vi "Migrate Common Dependencies.vi"(0 "project path":path, 5 "measurement path":path, 7 "dependencies path":path[](array[path]), 11 "error in":errorcluster) -> (4 "project reference":refnum<vi>, 6 "measurement core reference":refnum<vi>, 8 "outside items":string[](array[string]), 10 "library":T1[](array[typedef]), 15 "error out":errorcluster)   [LabVIEW 2021, in "Multiple Converter.lvlib"]
uses:
  Multiple Converter.lvlib
  TypeDefs/Library Info.ctl
  Path Functions/Path Functions.lvlib
  Converter Reusables/Converter Reusables.lvlib
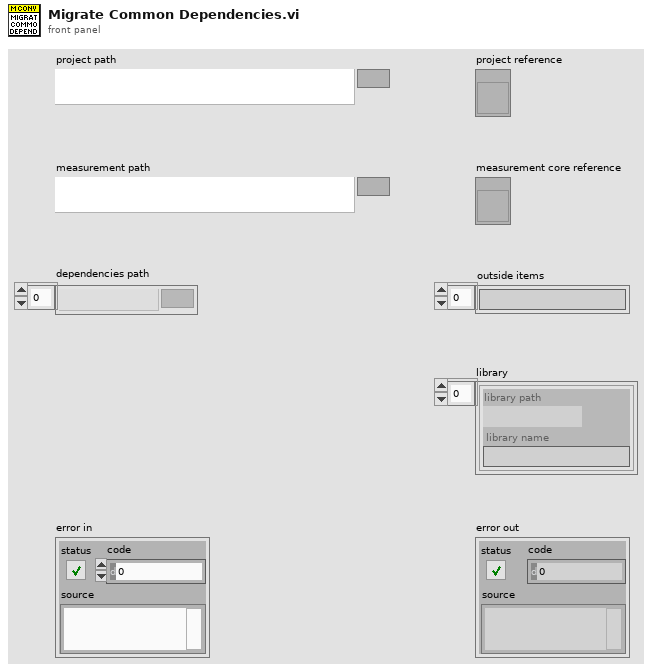
[diagram p1: front panel]
types:
  T1 = typedef "Multiple Converter.lvlib/Library Info.ctl" = cluster{"library path":path, "library name":string}
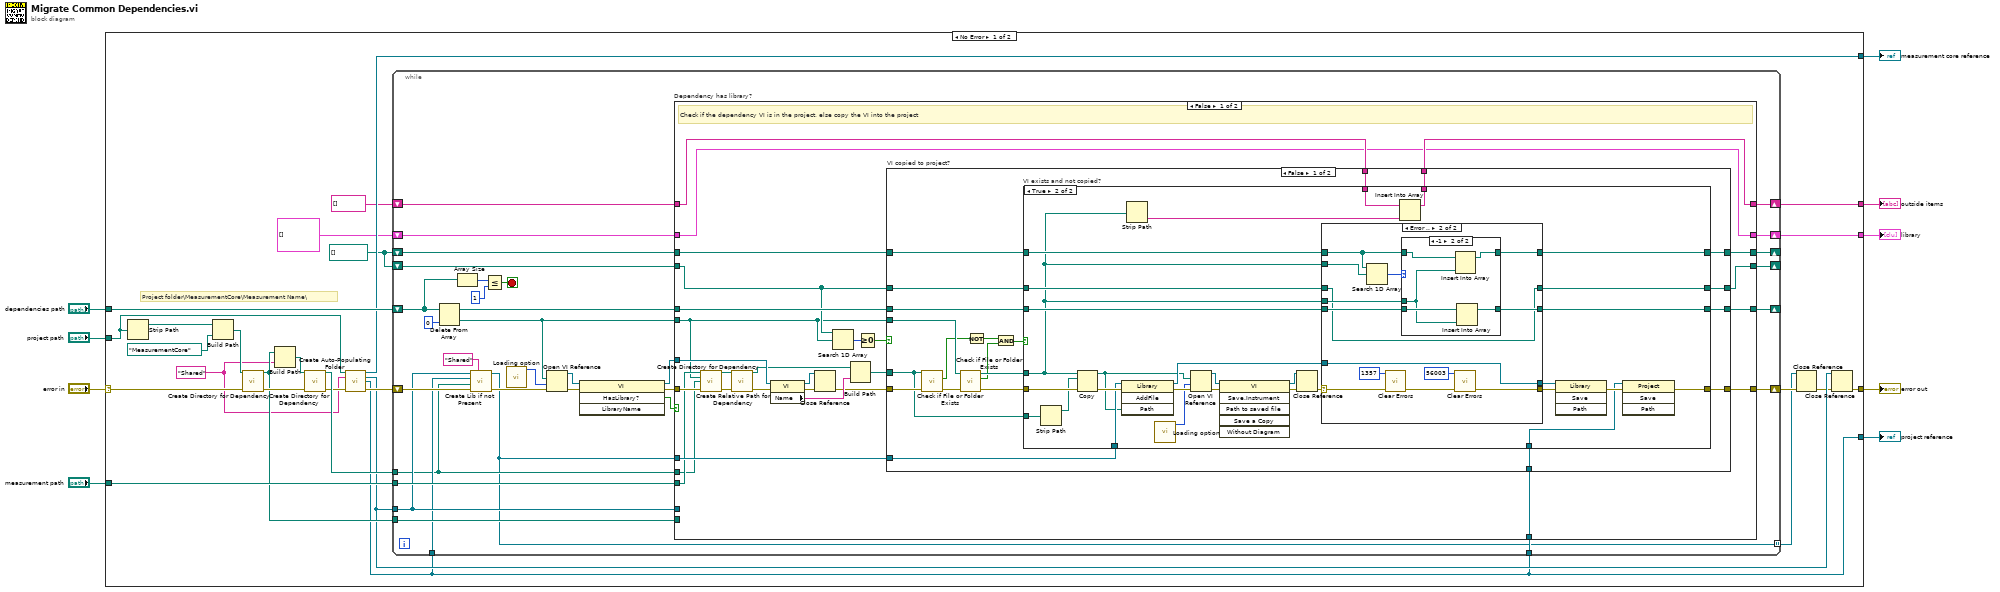
[diagram p0: block diagram]
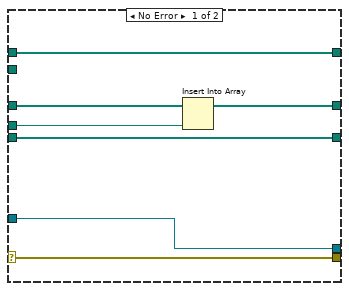
[diagram p3: hidden frame]
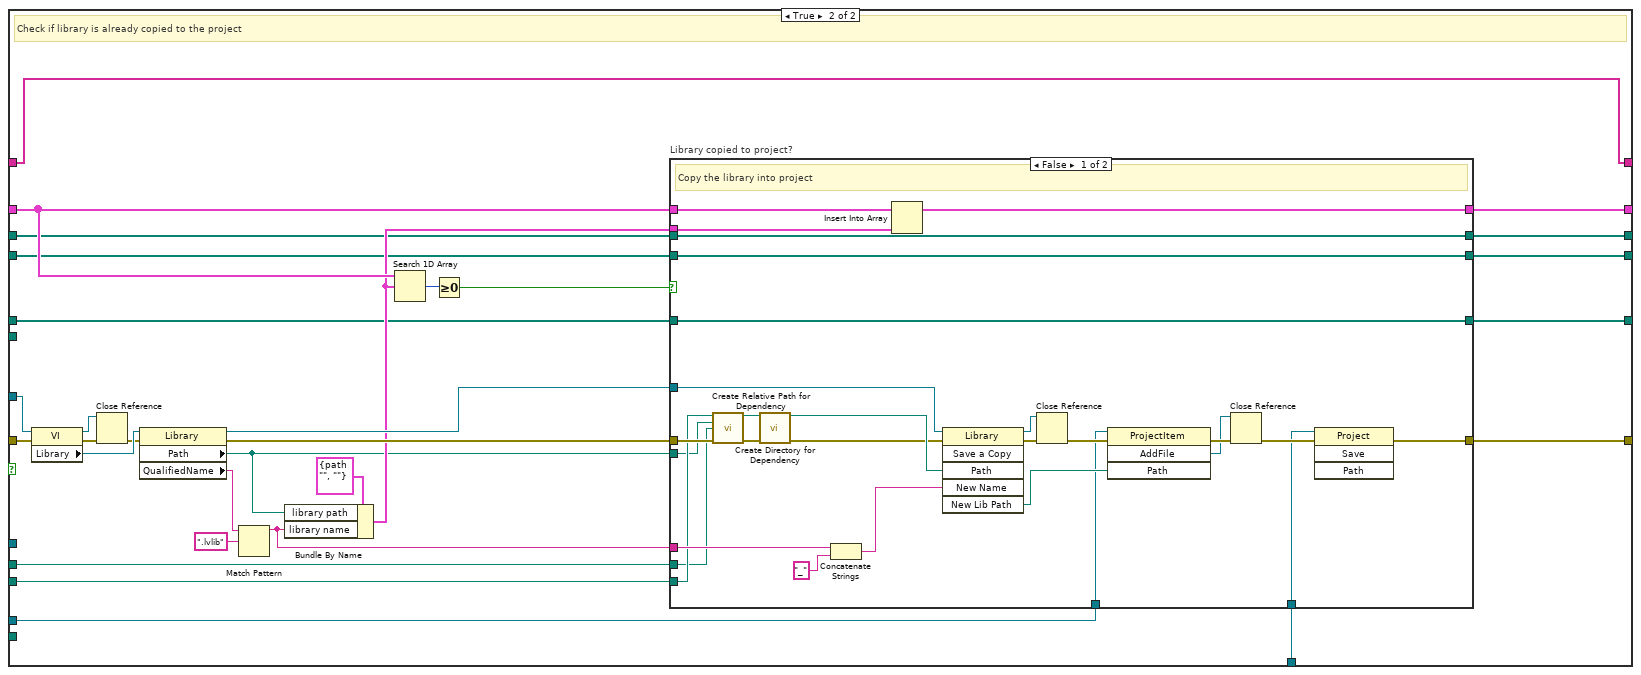
[diagram p6: hidden frame]
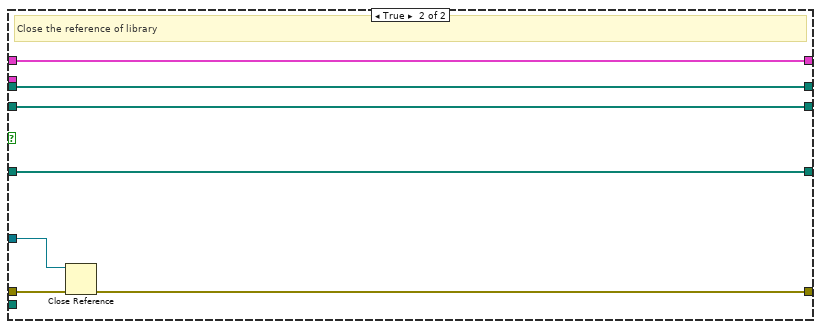
[diagram p7: hidden frame]
diagram:
  n1 = case shown="No Error" "error in" {
    selector: "error in" -> [w27 w250]
    tunnel: [w20 w250] -> w8
    tunnel: "project path" -> [w26 _]
    tunnel: "measurement path" -> [w31 _]
    tunnel: "dependencies path" -> [w35 _]
    tunnel: [w22 _] -> w4
    tunnel: [w16 _] -> w3
    tunnel: [w17 _] -> w2
    tunnel: [w10 _] -> w1
    frame No Error {
      w12 = "Shared"
      w13 = path[] []
      # "Project folder\\MeasurementCore\\Measurement Name\\"
      n2 = Strip Path(path=w26) -> (stripped path=w30:path)  [unwired: 1 out]
      n3 = Build Path(base path=w30, name or relative path=path "MeasurementCore") -> (appended path=w28:path)
      n4 = call "Create Directory for Dependency.vi"("directory path"=w28, "error in"=w27) -> ("directory path out"=w21:path, "error out"=w25:errorcluster)  [unwired: 12 in]
      n5 = Build Path(base path=w21, name or relative path=w12) -> (appended path=w34:path)
      n6 = call "Create Directory for Dependency.vi"("directory path"=w34, "error in"=w25) -> ("directory path out"=w33:path, "error out"=w24:errorcluster)  [unwired: 12 in]
      n7 = call "Create Auto-Populating Folder.vi"("project path"=w26, "plug-in name"=w12, "error in"=w24) -> ("measurement core reference"=w22:refnum<vi>, "folder reference"=w19:refnum<vi>, "project reference"=w16:refnum<vi>, "error out"=w23:errorcluster)  [unwired: 9 in]
      n8 = while {
        shift-right: [w57] -> w32
        shift-left: w23 -> [w46]
        shift-right: [w50] -> _
        shift-left: w35 -> [w66]
        tunnel: w33 -> [w42]
        shift-right: [w56] -> w10
        shift-left: T1[] [] -> [w59]
        tunnel: w31 -> [w55]
        shift-right: [w52] -> _
        shift-left: w13 -> [w53]
        tunnel: w21 -> [w49]
        tunnel: w19 -> [w44]
        shift-right: [w47] -> w17
        shift-left: string[] [] -> [w48]
        tunnel: w16 -> [w43]
        tunnel: w16 -> [w41]
        shift-right: [w40] -> _
        shift-left: w13 -> [w39]
        tunnel: [w38] -> w14 mode=indexing
        stop <- w65 stop-if-true
        n9 = Delete From Array(array=w66, index=0) -> (deleted portion=w54:path, array with subset deleted=w51:path[])  [unwired: 1 in]
        n10 = Array Size(array=w66) -> (size(s)=w68:i32)
        n11 = call "Create Lib if not Present.vi"("plug-in name"="Shared" ("Plug-in name"), "error in"=w46, "dest directory"=w42, "project ref"=w43, "virtual folder ref"=w44) -> ("error out"=w45:errorcluster, "library refnum"=w38:refnum<vi>)  [unwired: 5 in]
        n12 = Less Or Equal?(x=w68, y=1) -> (x <= y?=w65:bool)
        n13 = call "Loading option.vi"() -> ("options"=w36:i32)  [unwired: 11 in]
        n14 = Open VI Reference(vi path=w54, options=w36, error in (no error)=w45) -> (vi reference=w63:refnum<vi>, error out=w64:errorcluster)  [unwired: 3 in]
        n15 = invoke class="VI" method="HasLibrary?"(reference=w63, error in=w64) -> (reference out=w60:refnum<vi>, error out=w61:errorcluster, "Has Library?"=w62:bool)  [unwired: 2 in, 1 out]
        n16 = case "Dependency has library?" shown="False" w62 {
          tunnel: w61 -> [w74 w213]
          tunnel: w60 -> [w95 w214]
          tunnel: w59 -> [w78 w201]
          tunnel: [w90 w202] -> w57
          tunnel: [w78 w200] -> w56
          tunnel: w55 -> [w73 w198]
          tunnel: w42 -> [w71 w196]
          tunnel: w54 -> [w72 _]
          tunnel: w53 -> [w86 w193]
          tunnel: [w82 w192] -> w52
          tunnel: w51 -> [w89 w191]
          tunnel: [w88 w190] -> w50
          tunnel: w49 -> [_ _]
          tunnel: w44 -> [_ w189]
          tunnel: w48 -> [w80 w188]
          tunnel: [w79 w188] -> w47
          tunnel: w38 -> [w81 _]
          tunnel: w41 -> [w75 w187]
          tunnel: [w77 w185] -> w40
          tunnel: w39 -> [w76 w186]
          frame False {
            # "Check if the dependency VI is in the project, else copy the VI into the project"
            n17 = call "Create Relative Path for Dependency.vi"("old main path"=w73, "old dependency path"=w72, "new dir"=w71, "error in"=w74) -> ("directory"=w69:path, "error out"=w70:errorcluster)  [unwired: 10 in]
            n18 = call "Create Directory for Dependency.vi"("directory path"=w69, "error in"=w70) -> ("directory path out"=w87:path, "error out"=w96:errorcluster)  [unwired: 12 in]
            n19 = property class="VI"(reference=w95, error in=w96) -> (reference out=w91:refnum<vi>, error out=w94:errorcluster, "Name"=w93:string)
            n20 = Close Reference(reference=w91, error in (no error)=w94) -> (error out=w92:errorcluster)
            n21 = Search 1D Array(1D array=w86, element=w72) -> (index of element=w85:i32)  [unwired: 1 in]
            n22 = Build Path(base path=w87, name or relative path=w93) -> (appended path=w84:path)
            n23 = Greater Or Equal To 0?(x=w85) -> (x >= 0?=w83:bool)
            n24 = case "VI copied to project?" shown="False" w83 {
              tunnel: w92 -> [w117 w184]
              tunnel: w72 -> [w116 _]
              tunnel: [w113 w184] -> w90
              tunnel: w86 -> [w112 w183]
              tunnel: [w111 w183] -> w82
              tunnel: w84 -> [w107 _]
              tunnel: w89 -> [w110 w182]
              tunnel: [w109 w182] -> w88
              tunnel: w80 -> [w102 w181]
              tunnel: [w101 w181] -> w79
              tunnel: w81 -> [w100 _]
              tunnel: [w99 w180] -> w77
              tunnel: w76 -> [w98 w180]
              tunnel: w75 -> [w97 _]
              frame False {
                n25 = call <vilib>:"Check if File or Folder Exists.vi"("error in (no error)"=w117, "path"=w107) -> ("error out"=w108:errorcluster, "file or folder exists?"=w106:bool)  [unwired: 7 in, 1 out]
                n26 = call <vilib>:"Check if File or Folder Exists.vi"("error in (no error)"=w108, "path"=w116) -> ("error out"=w115:errorcluster, "file or folder exists?"=w104:bool, "dup path"=w114:path)  [unwired: 7 in]
                n27 = Not(x=w106) -> (.not. x?=w105:bool)
                n28 = And(x=w105, y=w104) -> (x .and. y?=w103:bool)
                n29 = case "VI exists and not copied?" shown="True" w103 {
                  tunnel: w115 -> [w122 w151]
                  tunnel: w114 -> [_ w131]
                  tunnel: [w122 w133] -> w113
                  tunnel: w112 -> [w121 w150]
                  tunnel: [w121 w149] -> w111
                  tunnel: w107 -> [_ w145]
                  tunnel: w110 -> [w120 w135]
                  tunnel: [w120 w134] -> w109
                  tunnel: w102 -> [w119 w144]
                  tunnel: [w119 w142] -> w101
                  tunnel: w100 -> [_ w141]
                  tunnel: [w118 w140] -> w99
                  tunnel: w98 -> [w118 w139]
                  tunnel: w97 -> [_ w132]
                  frame False {
                  }
                  frame True {
                    n30 = Strip Path(path=w145) -> (stripped path=w147:path)  [unwired: 1 out]
                    n31 = Copy(8:w151, 10:w147, 11:w131) -> (0:w148:errorcluster, 3:w129:path)  [unwired: 2 in, 1 out]
                    n32 = invoke class="Library" method="AddFile"(reference=w141, error in=w148, "Path"=w129) -> (reference out=w138:refnum<vi>, error out=w130:errorcluster)  [unwired: 1 in, 2 out]
                    n33 = Strip Path(path=w131) -> (name=w143:string)  [unwired: 1 out]
                    n34 = call "Loading option.vi"() -> ("options"=w123:i32)  [unwired: 11 in]
                    n35 = Open VI Reference(vi path=w129, options=w123, error in (no error)=w130) -> (vi reference=w128:refnum<vi>, error out=w124:errorcluster)  [unwired: 3 in]
                    n36 = invoke class="VI" method="Save.Instrument"(reference=w128, error in=w124) -> (reference out=w126:refnum<vi>, error out=w127:errorcluster)  [unwired: 4 in, 4 out]
                    n37 = Close Reference(reference=w126, error in (no error)=w127) -> (error out=w125:errorcluster)
                    n38 = case shown="Error .." w125 {
                      selector: w125 -> [w153 w172]
                      tunnel: w150 -> [w158 w159]
                      tunnel: [w157 w159] -> w149
                      tunnel: w131 -> [w156 w162]
                      tunnel: [w155 w163] -> w140
                      tunnel: w139 -> [w155 w164]
                      tunnel: [w154 w161] -> w136
                      tunnel: w138 -> [w154 w161]
                      tunnel: [w153 w170] -> w137
                      tunnel: w135 -> [w152 w166]
                      tunnel: [w152 w165] -> w134
                      tunnel: w131 -> [_ w167]
                      frame No Error {
                        n39 = Insert Into Array(array=w158, new element=w156) -> (w157:path[])  [unwired: 1 in]
                      }
                      frame Error {
                        n40 = Search 1D Array(1D array=w164, element=w167) -> (index of element=w160:i32)  [unwired: 1 in]
                        n41 = call <vilib>:"Clear Errors.vi"("error in (no error)"=w172, "specific error code to clear (0: all)"=1357) -> ("error out"=w171:errorcluster)  [unwired: 4 in, 1 out]
                        n42 = case shown="-1" w160 {
                          tunnel: w166 -> [w173 w179]
                          tunnel: [w173 w178] -> w165
                          tunnel: w164 -> [w174 w177]
                          tunnel: [w174 w176] -> w163
                          tunnel: w162 -> [_ w175]
                          frame Default {
                          }
                          frame -1 {
                            n43 = Insert Into Array(array=w177, new element=w175) -> (w176:path[])  [unwired: 1 in]
                            n44 = Insert Into Array(array=w179, new element=w175) -> (w178:path[])  [unwired: 1 in]
                          }
                        }
                        n45 = call <vilib>:"Clear Errors.vi"("error in (no error)"=w171, "specific error code to clear (0: all)"=56003) -> ("error out"=w170:errorcluster)  [unwired: 4 in, 1 out]
                      }
                    }
                    n46 = Insert Into Array(array=w144, new element=w143) -> (w142:string[])  [unwired: 1 in]
                    n47 = invoke class="Library" method="Save"(reference=w136, error in=w137) -> (error out=w146:errorcluster)  [unwired: 2 in, 3 out]
                    n48 = invoke class="Project" method="Save"(reference=w132, error in=w146) -> (error out=w133:errorcluster)  [unwired: 2 in, 3 out]
                  }
                }
              }
              frame True {
              }
            }
          }
          frame True {
            # "Check if library is already copied to the project"
            n49 = property class="VI"(reference=w214, error in=w213) -> (reference out=w204:refnum<vi>, error out=w212:errorcluster, "Library"=w211:refnum<vi>)
            n50 = Close Reference(reference=w204, error in (no error)=w212) -> (error out=w205:errorcluster)
            n51 = property class="Library"(reference=w211, error in=w205) -> (reference out=w203:refnum<vi>, error out=w206:errorcluster, "Path"=w197:path, "QualifiedName"=w207:string)
            n52 = Match Pattern(string=w207, regular expression=".lvlib") -> (before substring=w194:string)  [unwired: 1 in, 3 out]
            n53 = Bundle By Name(cluster=T1 {"library path"=path "", "library name"=""} ("Cluster"), "library path"=w197, "library name"=w194) -> (w199:T1)
            n54 = Search 1D Array(1D array=w201, element=w199) -> (index of element=w209:i32)  [unwired: 1 in]
            n55 = Greater Or Equal To 0?(x=w209) -> (x >= 0?=w208:bool)
            n56 = case "Library copied to project?" shown="False" w208 {
              tunnel: w206 -> [w219 w248]
              tunnel: w203 -> [w236 w249]
              tunnel: [w223 w247] -> w202
              tunnel: w201 -> [w242 w246]
              tunnel: [w241 w246] -> w200
              tunnel: w199 -> [w240 _]
              tunnel: w198 -> [w218 _]
              tunnel: w197 -> [w217 _]
              tunnel: w196 -> [w216 _]
              tunnel: w194 -> [w226 _]
              tunnel: w193 -> [w233 w245]
              tunnel: [w233 w245] -> w192
              tunnel: [w232 w244] -> w190
              tunnel: w191 -> [w232 w244]
              tunnel: w189 -> [w227 _]
              tunnel: w187 -> [w222 _]
              tunnel: [w221 w243] -> w185
              tunnel: w186 -> [w221 w243]
              frame False {
                # "Copy the library into project"
                n57 = call "Create Relative Path for Dependency.vi"("old main path"=w218, "old dependency path"=w217, "new dir"=w216, "error in"=w219) -> ("directory"=w215:path, "error out"=w220:errorcluster)  [unwired: 10 in]
                n58 = call "Create Directory for Dependency.vi"("directory path"=w215, "error in"=w220) -> ("directory path out"=w237:path, "error out"=w235:errorcluster)  [unwired: 12 in]
                n59 = Concatenate Strings(w226, "_" ("string")) -> (w224:string)
                n60 = Insert Into Array(array=w242, new element=w240) -> (w241:T1[])  [unwired: 1 in]
                n61 = invoke class="Library" method="Save a Copy"(reference=w236, error in=w235, "Path"=w237, "New Name"=w224) -> (reference out=w238:refnum<vi>, error out=w239:errorcluster, "New Lib Path"=w230:path)  [unwired: 2 in, 3 out]
                n62 = Close Reference(reference=w238, error in (no error)=w239) -> (error out=w234:errorcluster)
                n63 = invoke class="ProjectItem" method="AddFile"(reference=w227, error in=w234, "Path"=w230) -> (error out=w231:errorcluster, "AddFile"=w228:refnum<vi>)  [unwired: 1 in, 2 out]
                n64 = Close Reference(reference=w228, error in (no error)=w231) -> (error out=w229:errorcluster)
                n65 = invoke class="Project" method="Save"(reference=w222, error in=w229) -> (error out=w223:errorcluster)  [unwired: 2 in, 3 out]
              }
              frame True {
                # "Close the reference of library"
                n66 = Close Reference(reference=w249, error in (no error)=w248) -> (error out=w247:errorcluster)
              }
            }
          }
        }
      }
      n67 = Close Reference(reference=w14, error in (no error)=w32) -> (error out=w15:errorcluster)
      n68 = Close Reference(reference=w19, error in (no error)=w15) -> (error out=w20:errorcluster)
    }
    frame Error {
    }
  }
  "error out" <- w8
  "measurement core reference" <- w4
  "project reference" <- w3
  "outside items" <- w2
  "library" <- w1
